vi "LabVIEW Demo Station.vi"() -> ()   [LabVIEW 2020]
doc: "This template is for the Queued Message Handler design pattern.\n\nThe Event Handling Loop generates messages based on user interface actions.\n\nThe Message Handling Loop processes messages generated by the Event Handling Loop, or by other messages. The messages are string values, so new messages can be added easily to the Message Cases case structure in the Message Handling Loop. Each message cluster can also provide an optional value for Message Data, which is a variant that can be converted to whatever message-specific data is required."
uses:
  support/Demo_class/Demo.lvclass
  support/UI Data--cluster.ctl
  support/Message Queue/lvdemo_Message Queue.lvlib
  support/Message Queue/Enqueue Message (Single).vi
  support/Configuration--cluster.ctl
  support/Tree Tag to Demo--map.ctl
  <vilib>/Platform/browser.llb/Open URL in Default Browser (string).vi
panel:
  out "Title Text":string
  in  "Favorites Ring":u16(ring) items=["All Features", "DNatt's Favorites", "NORM!'s Favorites"]
  in  "Tree":string(tree)
  in  "Slideshow":bool
  in  "Back":bool
  in  "Try It":bool
  in  "Credits":string="The code for this demo station is available at https://demostation.dnatt.org"
  in  "Forward":bool
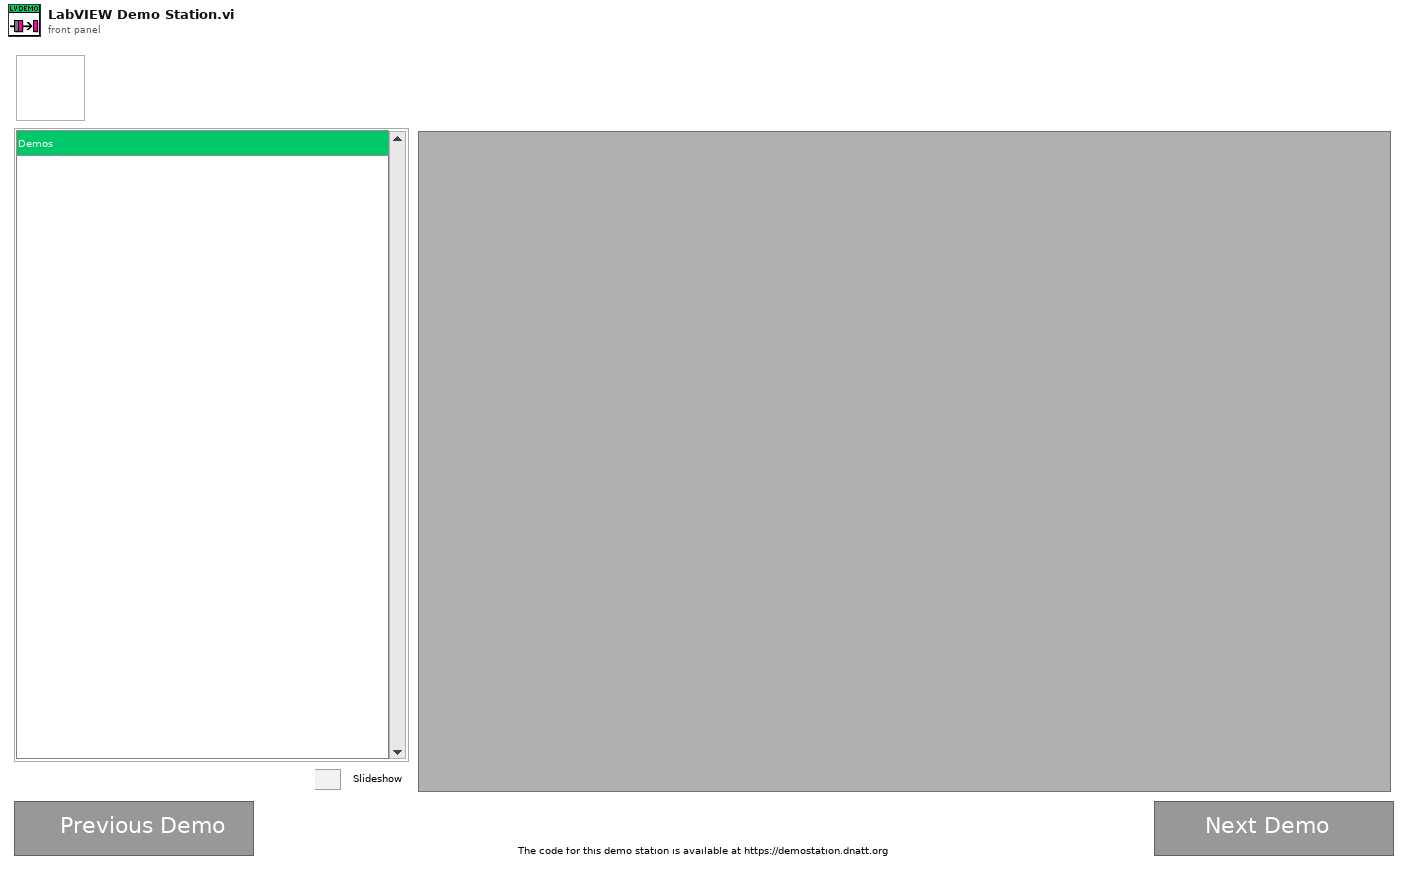
[diagram p1: front panel]
types:
  T1 = typedef "UI Data--cluster.ctl" = cluster{"Configuration":T2, "Start Timestamp":dbl, "Active Demos":T3, "Available Demos":T3}
  T2 = typedef "Configuration--cluster.ctl" = cluster{"Window Title":string, "Start Maximized":bool, "Slide Duration":i32, "Ignored Demos":string[], "Top Level Folder Order":string[], "Favorites":map{string, string[]}, "Show Favorites Ring":bool}
  T3 = typedef "Tree Tag to Demo--map.ctl" = map{string, refnum<class "Demo.lvclass">}
  T4 = typedef "lvdemo_Message Queue.lvlib/All Message Queues.ctl" = cluster{"UI":refnum<queue>}
  T5 = typedef "eventvkey.ctl" = enum16{"ASCII", "Enter", "Return", "Shift", "Ctrl", "Alt", "Cmd", "Opt", "Caps", "NumLock", "Clear", "Break", "Up", "Down", "Left", "Right", "Insert", "Delete", "Home", "End", "PageUp", "PageDown", "Escape", "Help", "Pause", "ScrollLock", "F1", "F2", "F3", "F4", "F5", "F6", "F7", "F8", "F9", "F10", "F11", "F12", "F13", "F14", "F15", "F16", "F17", "F18", "F19", "F20", "F21", "F22", "F23", "F24", "Play", "VolumeUp", "VolumeDown", "Mute", "Two Byte Char"}
  T6 = enum32{"Invalid", "Standard", "Closed", "Hidden", "Minimized", "Maximized"}
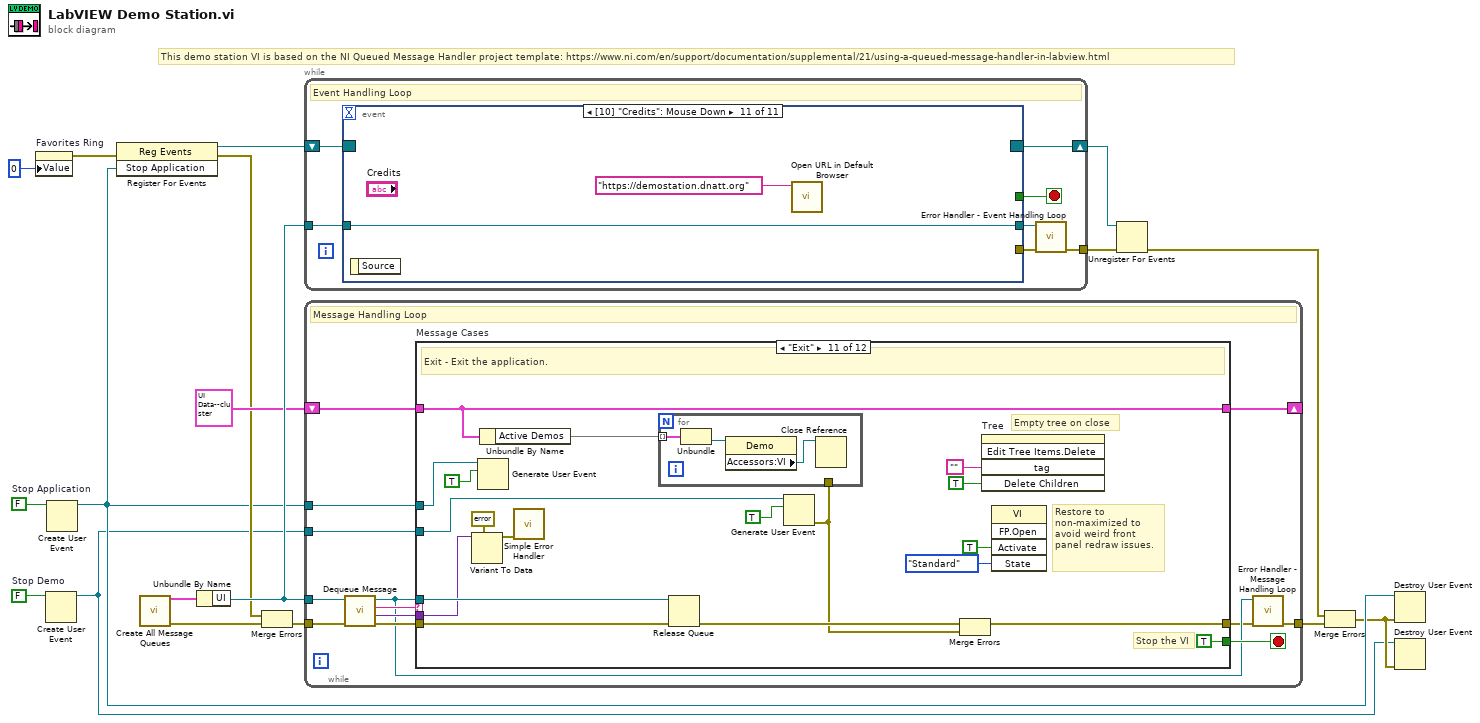
[diagram p0: block diagram]
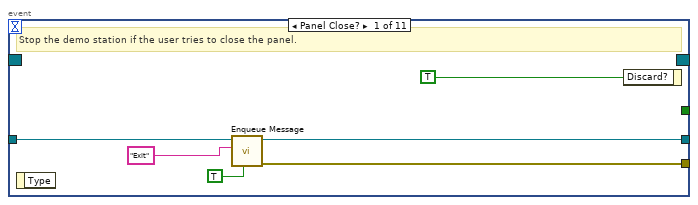
[diagram p2: hidden frame]
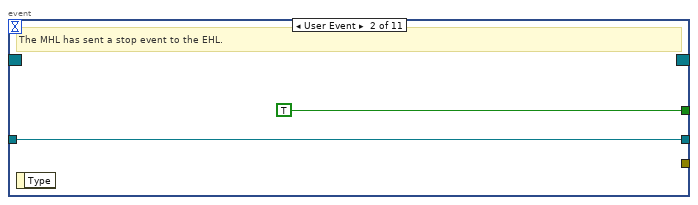
[diagram p3: hidden frame]
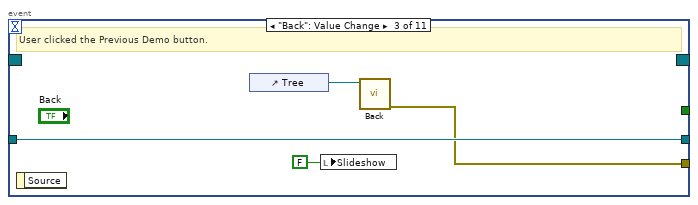
[diagram p4: hidden frame]
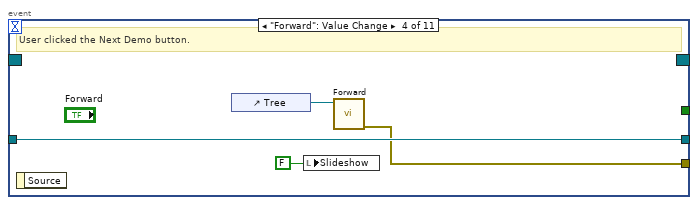
[diagram p5: hidden frame]
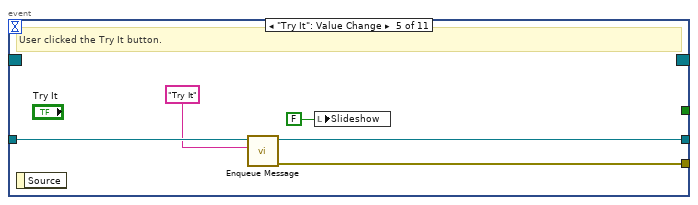
[diagram p6: hidden frame]
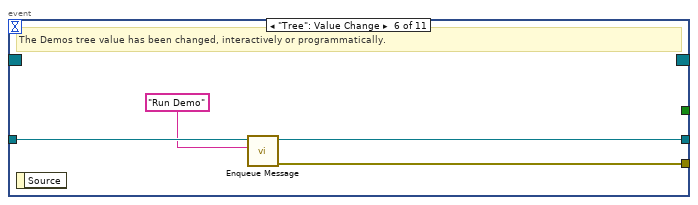
[diagram p7: hidden frame]
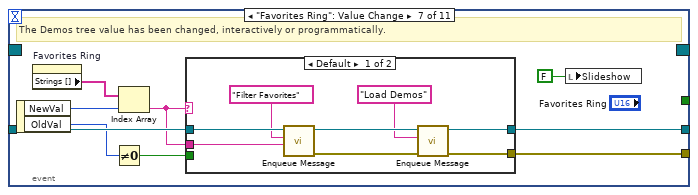
[diagram p8: hidden frame]
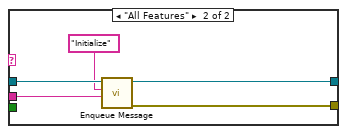
[diagram p9: hidden frame]
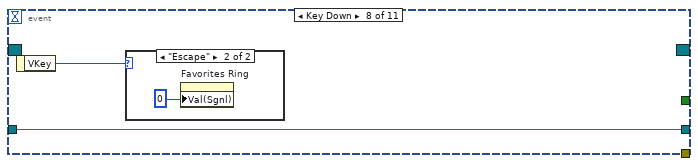
[diagram p10: hidden frame]
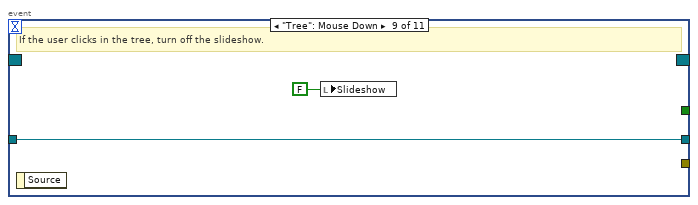
[diagram p12: hidden frame]
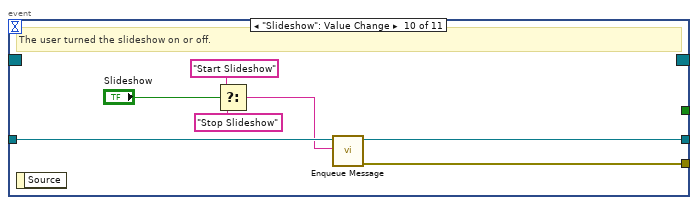
[diagram p13: hidden frame]
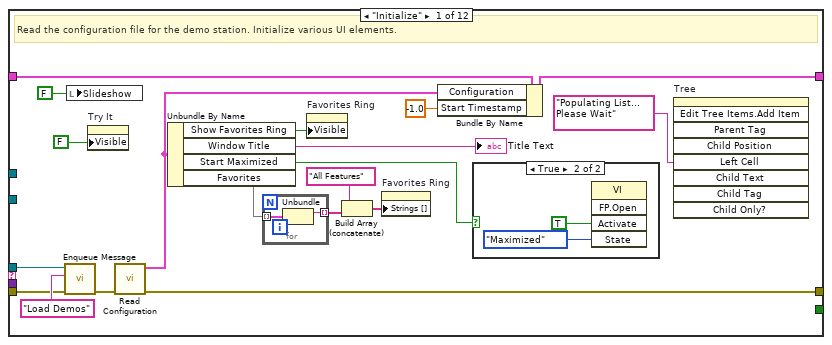
[diagram p14: hidden frame]
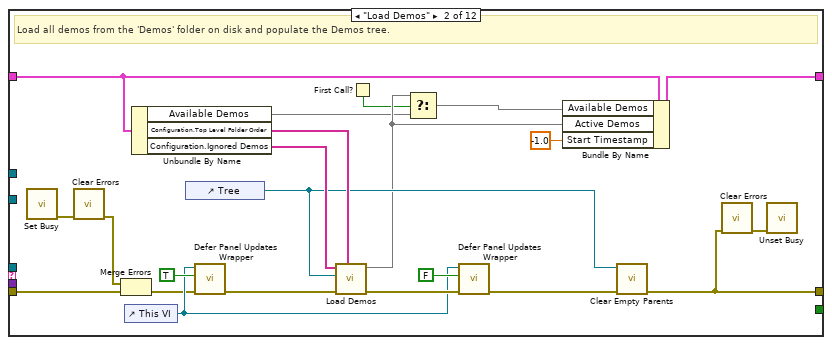
[diagram p16: hidden frame]
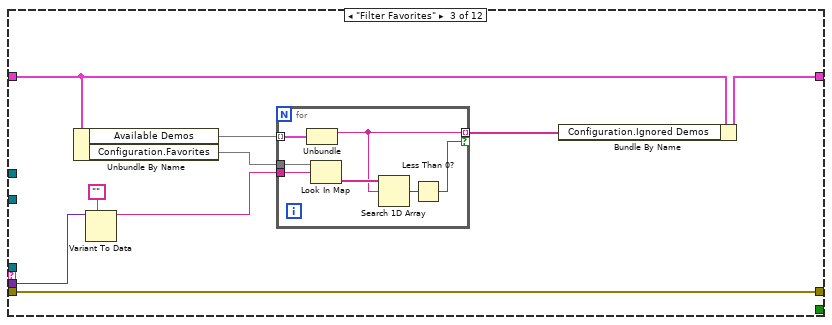
[diagram p17: hidden frame]
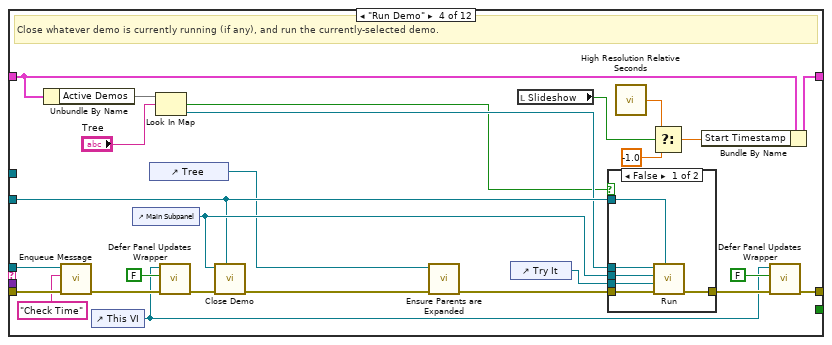
[diagram p18: hidden frame]
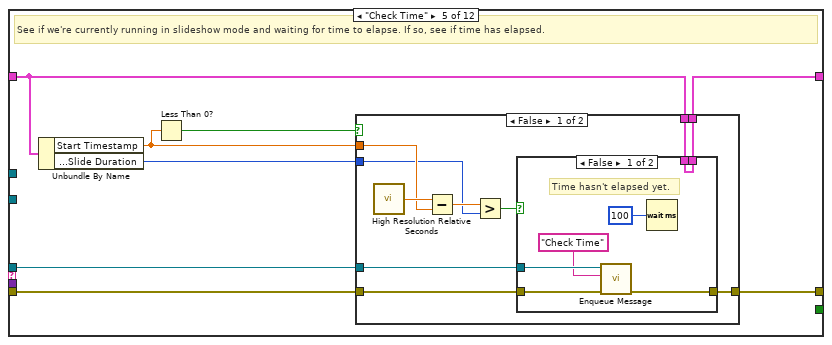
[diagram p20: hidden frame]
diagram:
  w5 = FALSE  # Stop Demo
  w7 = FALSE  # Stop Application
  # "This demo station VI is based on the NI Queued Message Handler project template: https://www.ni.com/en/support/documentation/supplemental/21/using-a-queued-message-handler-in-labview.html"
  n1 = property on="Favorites Ring" class="Ring (strict)"("Value"=u16 0 ("Value (Signaling)")) -> (error out=w1:errorcluster)  [unwired: 2 in, 1 out]
  n2 = Create User Event(user event datatype=w5) -> (user event=w3:refnum<user-event>)  [unwired: 1 in, 1 out]
  n3 = Create User Event(user event datatype=w7) -> (user event=w6:refnum<user-event>)  [unwired: 1 in, 1 out]
  n4 = register-events(error in=w1, w6) -> (reference out=w10:refnum<event-registration>, error out=w8:errorcluster)  [unwired: 1 in]
  n5 = call "Create All Message Queues.vi"() -> ("error out"=w18:errorcluster, "Message Queues out"=w17:T4)  [unwired: 10 in]
  n6 = Unbundle By Name(w17) -> ("UI"=w15:refnum<queue>)
  n7 = Merge Errors(w8, w18) -> (w9:errorcluster)
  n8 = while {
    tunnel: w15 -> [w25]
    shift-right: [w23] -> w13
    shift-left: w10 -> [w24]
    tunnel: [w19] -> w11
    stop <- w21 stop-if-true
    # "Event Handling Loop"
    n9 = event shown="[10] \"Credits\": Mouse Down" {
      selector: w24 -> [_ _ _ _ _ _ _ _ _ _ _]
      dyn-events: [_ _ _ _ _ _ _ _ _ _ _] -> w23
      timeout: _ -> [_ _ _ _ _ _ _ _ _ _ _]
      tunnel: [_ TRUE ("Discard?") _ _ _ _ _ _ _ _ _] -> w21
      tunnel: w25 -> [w30 w33 w37 w41 w46 w50 w59 w74 w77 w84 w86]
      tunnel: [w29 _ w35 w39 w44 w48 w58 _ _ w80 _] -> w22
      tunnel: [w28 w33 w37 w41 w45 w49 w57 w74 w77 w81 w86] -> w20
      event Panel Close? {
        # "Stop the demo station if the user tries to close the panel."
        n10 = event-data() -> ()  [unwired: 1 in, 1 out]
        n11 = call-poly "Enqueue Message.vi"("Priority Message? (F)"=TRUE, "Message"="Exit", "Message Queue"=w30) -> ("error out"=w29:errorcluster, "dup Message Queue"=w28:refnum<queue>)  [unwired: 7 in]
        n12 = event-data("Discard?"=TRUE) -> ()  [unwired: 1 in, 1 out]
      }
      event User Event {
        # "The MHL has sent a stop event to the EHL."
        n13 = event-data() -> ()  [unwired: 1 in, 1 out]
      }
      event "Back": Value Change {
        # "User clicked the Previous Demo button."
        n14 = event-data() -> ()  [unwired: 1 in, 1 out]
        n15 = control-ref of="Tree"() -> (w36:refnum<vi>)
        n16 = local write "Slideshow"(FALSE ("Slideshow")) -> ()
        n17 = call "Back.vi"("Tree"=w36) -> ("error out"=w35:errorcluster)  [unwired: 10 in]
      }
      event "Forward": Value Change {
        # "User clicked the Next Demo button."
        n18 = event-data() -> ()  [unwired: 1 in, 1 out]
        n19 = control-ref of="Tree"() -> (w40:refnum<vi>)
        n20 = local write "Slideshow"(FALSE ("Slideshow")) -> ()
        n21 = call "Forward.vi"("Tree"=w40) -> ("error out"=w39:errorcluster)  [unwired: 10 in]
      }
      event "Try It": Value Change {
        # "User clicked the Try It button."
        n22 = event-data() -> ()  [unwired: 1 in, 1 out]
        n23 = call-poly "Enqueue Message.vi"("Message"="Try It", "Message Queue"=w46) -> ("error out"=w44:errorcluster, "dup Message Queue"=w45:refnum<queue>)  [unwired: 8 in]
        n24 = local write "Slideshow"(FALSE ("Slideshow")) -> ()
      }
      event "Tree": Value Change {
        # "The Demos tree value has been changed, interactively or programmatically."
        n25 = event-data() -> ()  [unwired: 1 in, 1 out]
        n26 = call-poly "Enqueue Message.vi"("Message"="Run Demo", "Message Queue"=w50) -> ("error out"=w48:errorcluster, "dup Message Queue"=w49:refnum<queue>)  [unwired: 8 in]
      }
      event "Favorites Ring": Value Change {
        # "The Demos tree value has been changed, interactively or programmatically."
        n27 = event-data() -> ("NewVal"=w54:u16, "OldVal"=w52:u16)  [unwired: 1 in]
        n28 = property on="Favorites Ring" class="Ring (strict)"() -> ("Strings []"=w55:string[])  [unwired: 2 in, 2 out]
        n29 = Not Equal To 0?(x=w52) -> (x != 0?=w51:bool)
        n30 = Index Array(array=w55, index=w54) -> (element=w53:string)
        n31 = case shown="Default" w53 {
          tunnel: w59 -> [w61 w72]
          tunnel: [w65 w69] -> w58
          tunnel: [w64 w70] -> w57
          tunnel: w53 -> [w62 w68]
          tunnel: w51 -> [_ _]
          frame Default {
            n32 = call-poly "Enqueue Message.vi"("Message Data"=w62, "Message"="Filter Favorites", "Message Queue"=w61) -> ("error out"=w66:errorcluster, "dup Message Queue"=w67:refnum<queue>)  [unwired: 7 in]
            n33 = call-poly "Enqueue Message.vi"("error in (no error)"=w66, "Message"="Load Demos", "Message Queue"=w67) -> ("error out"=w65:errorcluster, "dup Message Queue"=w64:refnum<queue>)  [unwired: 7 in]
          }
          frame "All Features" {
            n34 = call-poly "Enqueue Message.vi"("Message Data"=w68, "Message"="Initialize", "Message Queue"=w72) -> ("error out"=w69:errorcluster, "dup Message Queue"=w70:refnum<queue>)  [unwired: 7 in]
          }
        }
        n35 = local write "Slideshow"(FALSE ("Slideshow")) -> ()
      }
      event Key Down {
        n36 = event-data() -> ("VKey"=w73:T5)  [unwired: 1 in]
        n37 = case shown="\"Escape\"" w73 {
          frame Default {
          }
          frame "Escape" {
            n38 = property on="Favorites Ring" class="Ring (strict)"("Val(Sgnl)"=u16 0 ("Value (Signaling)")) -> ()  [unwired: 2 in, 2 out]
          }
        }
      }
      event "Tree": Mouse Down {
        # "If the user clicks in the tree, turn off the slideshow."
        n39 = event-data() -> ()  [unwired: 1 in, 1 out]
        n40 = local write "Slideshow"(FALSE ("Slideshow")) -> ()
      }
      event "Slideshow": Value Change {
        # "The user turned the slideshow on or off."
        n41 = event-data() -> ()  [unwired: 1 in, 1 out]
        n42 = Select(t="Start Slideshow", s="Slideshow", f="Stop Slideshow") -> (s? t:f=w78:string)
        n43 = call-poly "Enqueue Message.vi"("Message"=w78, "Message Queue"=w84) -> ("error out"=w80:errorcluster, "dup Message Queue"=w81:refnum<queue>)  [unwired: 8 in]
      }
      event "Credits": Mouse Down {
        n44 = event-data() -> ()  [unwired: 1 in, 1 out]
        n45 = call-poly <vilib>:"Open URL in Default Browser.vi"("URL"="https://demostation.dnatt.org") -> ()  [unwired: 5 in, 2 out]
      }
    }
    n46 = call "Error Handler - Event Handling Loop.vi"("error in (no error)"=w22, "Message Queue"=w20) -> ("dup error in"=w19:errorcluster)  [unwired: 8 in, 1 out]
  }
  n47 = while {
    tunnel: w15 -> [w91]
    shift-right: [w98] -> _
    shift-left: T1 {"Configuration"={"Window Title"="", "Start Maximized"=FALSE, "Slide Duration"=0, "Ignored Demos"=[], "Top Level Folder Order"=[], "Favorites"={}, "Show Favorites Ring"=FALSE}, "Start Timestamp"=0.0, "Active Demos"={}, "Available Demos"={}} ("Data Cluster") -> [w99]
    tunnel: w6 -> [w96]
    tunnel: w9 -> [w95]
    tunnel: [w89] -> w16
    tunnel: w3 -> [w87]
    stop <- w97 stop-if-true
    # "Message Handling Loop"
    n48 = call "Dequeue Message.vi"("error in (no error)"=w95, "Message Queue"=w91) -> ("error out"=w94:errorcluster, "Message Data"=w92:variant, "Message"=w93:string, "dup Message Queue"=w90:refnum<queue>)  [unwired: 6 in]
    n49 = case "Message Cases" shown="\"Exit\"" w93 {
      selector: w93 -> [_ _ _ _ _ _ _ _ _ _ _ w280]
      tunnel: w90 -> [w113 _ _ w185 w198 _ _ _ _ _ w273 _]
      tunnel: w94 -> [w111 w141 w153 w186 w197 w229 w238 w244 w251 w254 w269 _]
      tunnel: [w109 w128 w153 w172 w196 w230 w237 w244 w245 w252 w270 w277] -> w88
      tunnel: w99 -> [w118 w130 w152 w181 w194 w233 w239 w243 w250 w253 w264 w283]
      tunnel: [w117 w144 w146 w180 w195 w235 w239 w242 w250 w253 w264 w283] -> w98
      tunnel: [_ _ _ _ _ _ _ _ _ _ TRUE _] -> w97
      tunnel: w92 -> [_ _ w149 _ _ _ _ _ w249 _ w266 _]
      tunnel: w96 -> [_ _ _ _ _ _ _ _ _ _ w262 _]
      tunnel: w87 -> [_ _ _ w179 _ _ _ _ _ _ w259 _]
      frame "Initialize" {
        # "Read the configuration file for the demo station. Initialize various UI elements."
        n50 = call-poly "Enqueue Message.vi"("error in (no error)"=w111, "Message"="Load Demos", "Message Queue"=w113) -> ("error out"=w110:errorcluster)  [unwired: 7 in, 1 out]
        n51 = local write "Slideshow"(FALSE ("Demo Mode")) -> ()
        n52 = property on="Try It" class="Bool"("Visible"=FALSE) -> ()  [unwired: 2 in, 2 out]
        n53 = call "Read Configuration.vi"("error in"=w110) -> ("error out"=w109:errorcluster, "Configuration"=w116:T2)  [unwired: 9 in]
        n54 = Unbundle By Name(w116) -> ("Show Favorites Ring"=w100:bool, "Window Title"=→"Title Text":string, "Start Maximized"=w114:bool, "Favorites"=w104:map{string, string[]})
        n55 = for {
          tunnel: w104 -> [w120] mode=indexing
          tunnel: [w119] -> w103 mode=indexing
          n56 = Unbundle(w120) -> ("key"=w119:string)  [unwired: 1 out]
        }
        n57 = property on="Favorites Ring" class="Ring (strict)"("Visible"=w100) -> ()  [unwired: 2 in, 2 out]
        n58 = Build Array (concatenate)("All Features", w103) -> (w101:string[])
        n59 = property on="Favorites Ring" class="Ring (strict)"("Strings []"=w101) -> ()  [unwired: 2 in, 2 out]
        n60 = Bundle By Name(cluster=w118, "Configuration"=w116, "Start Timestamp"=-1.0) -> (w117:T1)
        n61 = case shown="True" w114 {
          frame False {
          }
          frame True {
            n62 = invoke class="VI" method="FP.Open"("Activate"=TRUE ("Activate?"), "State"=T6."Maximized") -> ()  [unwired: 3 in, 5 out]
          }
        }
        n63 = invoke on="Tree" class="Tree (strict)" method="Edit Tree Items.Add Item"("Left Cell"="Populating List... Please Wait") -> ()  [unwired: 8 in, 9 out]
      }
      frame "Load Demos" {
        # "Load all demos from the 'Demos' folder on disk and populate the Demos tree."
        n64 = call <vilib>:"Set Busy.vi"() -> ("error out"=w135:errorcluster)  [unwired: 10 in, 1 out]
        n65 = call <vilib>:"Clear Errors.vi"("error in (no error)"=w135) -> ("error out"=w133:errorcluster)  [unwired: 5 in, 1 out]
        n66 = Merge Errors(w133, w141) -> (w134:errorcluster)
        n67 = control-ref of="This VI"() -> (w136:refnum<vi>)
        n68 = Unbundle By Name(w130) -> ("Available Demos"=w125:T3, "Configuration.Top Level Folder Order"=w131:string[], "Configuration.Ignored Demos"=w142:string[])
        n69 = control-ref of="Tree"() -> (w127:refnum<vi>)
        n70 = call "Defer Panel Updates Wrapper.vi"("error in"=w134, "Defer Updates"=TRUE, "VI"=w136) -> ("error out"=w140:errorcluster)  [unwired: 8 in]
        n71 = call "Load Demos.vi"("Top Level Folder Order"=w131, "error in"=w140, "Tree"=w127, "Ignored Demos"=w142) -> ("error out"=w139:errorcluster, "Demos"=w126:T3)  [unwired: 6 in]
        n72 = First Call?() -> (First Call?: T/F=w123:bool)
        n73 = Select(t=w126, s=w123, f=w125) -> (s? t:f=w124:T3)
        n74 = call "Defer Panel Updates Wrapper.vi"("error in"=w139, "Defer Updates"=FALSE, "VI"=w136) -> ("error out"=w129:errorcluster)  [unwired: 8 in]
        n75 = Bundle By Name(cluster=w130, "Available Demos"=w124, "Active Demos"=w126, "Start Timestamp"=-1.0) -> (w144:T1)
        n76 = call "Clear Empty Parents.vi"("error in (no error)"=w129, "TreeControl in"=w127) -> ("error IO"=w128:errorcluster)  [unwired: 9 in]
        n77 = call <vilib>:"Clear Errors.vi"("error in (no error)"=w128) -> ("error out"=w132:errorcluster)  [unwired: 5 in, 1 out]
        n78 = call <vilib>:"Unset Busy.vi"("error in (no error)"=w132) -> ()  [unwired: 10 in, 1 out]
      }
      frame "Filter Favorites" {
        n79 = Unbundle By Name(w152) -> ("Available Demos"=w151:T3, "Configuration.Favorites"=w150:map{string, string[]})
        n80 = Variant To Data(type="", Variant=w149) -> (data=w147:string)  [unwired: 1 in, 1 out]
        n81 = for {
          tunnel: w151 -> [w160] mode=indexing
          tunnel: w150 -> [w159]
          tunnel: w147 -> [w158]
          tunnel: [w155] -> w145 mode=indexing if=w154
          n82 = Unbundle(w160) -> ("Tree Tag"=w155:string)  [unwired: 1 out]
          n83 = Look In Map(map=w159, key=w158) -> (value=w157:string[])  [unwired: 1 in, 1 out]
          n84 = Search 1D Array(1D array=w157, element=w155) -> (index of element=w156:i32)  [unwired: 1 in]
          n85 = Less Than 0?(x=w156) -> (x < 0?=w154:bool)
        }
        n86 = Bundle By Name(cluster=w152, "Configuration.Ignored Demos"=w145) -> (w146:T1)
      }
      frame "Run Demo" {
        # "Close whatever demo is currently running (if any), and run the currently-selected demo."
        n87 = Unbundle By Name(w181) -> ("Active Demos"=w178:T3)
        n88 = call-poly "Enqueue Message.vi"("error in (no error)"=w186, "Message"="Check Time", "Message Queue"=w185) -> ("error out"=w175:errorcluster)  [unwired: 7 in, 1 out]
        n89 = control-ref of="This VI"() -> (w169:refnum<vi>)
        n90 = control-ref of="Main Subpanel"() -> (w184:refnum<vi>)
        n91 = control-ref of="Tree"() -> (w165:refnum<vi>)
        n92 = Look In Map(map=w178, key="Tree") -> (key not found?=w168:bool, value=w176:refnum<class "Demo.lvclass">)  [unwired: 1 in]
        n93 = call "Defer Panel Updates Wrapper.vi"("error in"=w175, "Defer Updates"=FALSE, "VI"=w169) -> ("error out"=w174:errorcluster)  [unwired: 8 in]
        n94 = call "Close Demo.vi"("Stop Demo"=w179, "error in"=w174, "Main Subpanel"=w184) -> ("error out"=w167:errorcluster)  [unwired: 8 in]
        n95 = call "Ensure Parents are Expanded.vi"("error in"=w167, "Tree"=w165) -> ("error out"=w166:errorcluster)  [unwired: 9 in]
        n96 = control-ref of="Try It"() -> (w182:refnum<vi>)
        n97 = local read "Slideshow"() -> (w162:bool)
        n98 = case shown="False" w168 {
          tunnel: w166 -> [w192 w193]
          tunnel: w184 -> [w191 _]
          tunnel: w182 -> [w190 _]
          tunnel: w179 -> [w189 _]
          tunnel: w176 -> [w188 _]
          tunnel: [w187 w193] -> w173
          frame False {
            n99 = call-dynamic "Run.vi"("Stop Demo"=w189, "error in"=w192, "Try It Button"=w190, "Main Subpanel"=w191, "Demo in"=w188) -> ("error out"=w187:errorcluster)  [unwired: 5 in, 1 out]
          }
          frame True {
          }
        }
        n100 = call <vilib>:"High Resolution Relative Seconds.vi"() -> ("relative seconds"=w164:dbl)
        n101 = Select(t=w164, s=w162, f=-1.0) -> (s? t:f=w163:dbl)
        n102 = Bundle By Name(cluster=w181, "Start Timestamp"=w163) -> (w180:T1)
        n103 = call "Defer Panel Updates Wrapper.vi"("error in"=w173, "Defer Updates"=FALSE, "VI"=w169) -> ("error out"=w172:errorcluster)  [unwired: 8 in]
      }
      frame "Check Time" {
        # "See if we're currently running in slideshow mode and waiting for time to elapse. If so, see if time has elapsed."
        n104 = Unbundle By Name(w194) -> ("Start Timestamp"=w200:dbl, "Configuration.Slide Duration"=w199:i32)
        n105 = Less Than 0?(x=w200) -> (x < 0?=w201:bool)
        n106 = case shown="False" w201 {
          tunnel: w200 -> [w210 _]
          tunnel: w199 -> [w208 _]
          tunnel: w198 -> [w205 _]
          tunnel: w197 -> [w207 w225]
          tunnel: [w206 w225] -> w196
          tunnel: w194 -> [w203 w224]
          tunnel: [w202 w224] -> w195
          frame False {
            n107 = call <vilib>:"High Resolution Relative Seconds.vi"() -> ("relative seconds"=w211:dbl)
            n108 = Subtract(x=w211, y=w210) -> (x-y=w209:dbl)
            n109 = Greater?(x=w209, y=w208) -> (0:w204:bool)
            n110 = case shown="False" w204 {
              tunnel: w207 -> [w216 w219]
              tunnel: [w215 w220] -> w206
              tunnel: w205 -> [w214 _]
              tunnel: w203 -> [w212 w223]
              tunnel: [w212 w222] -> w202
              frame False {
                # "Time hasn't elapsed yet."
                n111 = call-poly "Enqueue Message.vi"("error in (no error)"=w216, "Message"="Check Time", "Message Queue"=w214) -> ("error out"=w215:errorcluster)  [unwired: 7 in, 1 out]
                n112 = Wait (ms)(milliseconds to wait=u32 100) -> ()  [unwired: 1 out]
              }
              frame True {
                # "Time elapsed. Go to next demo."
                n113 = control-ref of="Tree"() -> (w218:refnum<vi>)
                n114 = Bundle By Name(cluster=w223, "Start Timestamp"=-1.0) -> (w222:T1)
                n115 = call "Forward.vi"("error in"=w219, "Tree"=w218) -> ("error out"=w220:errorcluster)  [unwired: 9 in]
              }
            }
          }
          frame True {
            # "No timestamp stored, don't check"
          }
        }
      }
      frame "Try It" {
        # "Execute the 'Try It' code for the current demo."
        n116 = Unbundle By Name(w233) -> ("Active Demos"=w232:T3)
        n117 = local read "Tree"() -> (w231:string)
        n118 = Look In Map(map=w232, key=w231) -> (value=w228:refnum<class "Demo.lvclass">)  [unwired: 1 in, 1 out]
        n119 = control-ref of="This VI"() -> (w227:refnum<vi>)
        n120 = call "Try It.vi"("error in"=w229, "Main Demo UI"=w227, "Demo"=w228) -> ("error out"=w230:errorcluster)  [unwired: 8 in]
        n121 = local write "Slideshow"(FALSE ("Slideshow")) -> ()
        n122 = Bundle By Name(cluster=w233, "Start Timestamp"=-1.0) -> (w235:T1)
      }
      frame "Start Slideshow" {
        # "Start the slideshow."
        n123 = control-ref of="Tree"() -> (w236:refnum<vi>)
        n124 = call "Forward.vi"("error in"=w238, "Tree"=w236) -> ("error out"=w237:errorcluster)  [unwired: 9 in]
      }
      frame "Stop Slideshow" {
        # "Stop slideshow."
        n125 = Bundle By Name(cluster=w243, "Start Timestamp"=-1.0) -> (w242:T1)
        n126 = local write "Slideshow"(FALSE ("Slideshow")) -> ()
      }
      frame "Error" {
        # "Display an error dialog. This message is sent by the \"Error Handler\" VIs at the end of other loops in this application."
        n127 = Variant To Data(error in=w251, type=errorcluster {"status"=FALSE, "code"=0, "source"=""} ("error constant"), Variant=w249) -> (data=w247:errorcluster, error out=w246:errorcluster)
        n128 = call <vilib>:"Simple Error Handler.vi"("error in (no error)"=w247) -> ()  [unwired: 4 in, 5 out]
        n129 = Merge Errors(w246) -> (w245:errorcluster)
      }
      frame "---Copy This Frame---" {
        # "Duplicate this frame when creating new messages.  Change this comment in the duplicated frame to describe this message."
        n130 = Merge Errors(w254) -> (w252:errorcluster)
      }
      frame "Exit" {
        # "Restore to non-maximized to avoid weird front panel redraw issues."
        # "Empty tree on close"
        # "Stop the VI"
        # "Exit - Exit the application."
        n131 = Variant To Data(type=errorcluster {"status"=FALSE, "code"=0, "source"=""} ("error constant"), Variant=w266) -> (data=w267:errorcluster)  [unwired: 1 in, 1 out]
        n132 = Generate User Event(user event=w262, event data cluster=TRUE ("event data")) -> ()  [unwired: 2 in, 2 out]
        n133 = Unbundle By Name(w264) -> ("Active Demos"=w263:T3)
        n134 = call <vilib>:"Simple Error Handler.vi"("error in (no error)"=w267) -> ()  [unwired: 4 in, 5 out]
        n135 = Release Queue(queue=w273, error in (no error)=w269) -> (error out=w271:errorcluster)  [unwired: 1 in, 2 out]
        n136 = Generate User Event(user event=w259, event data cluster=TRUE ("event data")) -> (error out=w260:errorcluster)  [unwired: 2 in, 1 out]
        n137 = for {
          tunnel: w263 -> [w276] mode=indexing
          tunnel: w260 -> [_]
          n138 = Unbundle(w276) -> ("Demo"=w274:refnum<class "Demo.lvclass">)  [unwired: 1 out]
          n139 = property class="Demo"(reference=w274) -> ("Accessors:VI"=w275:refnum<vi>)  [unwired: 1 in, 2 out]
          n140 = Close Reference(reference=w275) -> ()  [unwired: 1 in, 1 out]
        }
        n141 = Merge Errors(w271, w260) -> (w270:errorcluster)
        n142 = invoke on="Tree" class="Tree (strict)" method="Edit Tree Items.Delete"("tag"="", "Delete Children"=TRUE) -> ()  [unwired: 3 in, 5 out]
        n143 = invoke class="VI" method="FP.Open"("Activate"=TRUE ("Activate?"), "State"=T6."Standard") -> ()  [unwired: 3 in, 5 out]
      }
      frame Default {
        # "'Default' case only runs if there is a message that isn't defined in any of the other cases.  Output a programming error."
        n144 = Format Into String(format string="The invalid message string \"%s\" was received in the Message Handling Loop.", w280) -> (resulting string=w278:string)  [unwired: 2 in, 1 out]
        n145 = call <vilib>:"Error Cluster From Error Code.vi"("show call chain? (False)"=TRUE, "error message (\"\")"=w278, "error code (0)"=1) -> ("error out"=w277:errorcluster)  [unwired: 6 in]
      }
    }
    n146 = call "Error Handler - Message Handling Loop.vi"("error in (no error)"=w88, "Message Queue"=w90) -> ("dup error in"=w89:errorcluster)  [unwired: 8 in, 1 out]
  }
  n147 = Unregister For Events(event registration refnum=w13, error in=w11) -> (error out=w14:errorcluster)
  n148 = Merge Errors(w14, w16) -> (w4:errorcluster)
  n149 = Destroy User Event(user event=w6, error in=w4) -> ()  [unwired: 1 out]
  n150 = Destroy User Event(user event=w3, error in=w4) -> ()  [unwired: 1 out]
